vi "work1_GetOrder.vi"() -> ()   [LabVIEW 2026]
panel:
  out "Client order":i32
  out "Order ID":i32
  in  "ID":i32
  in  "stop 2":bool
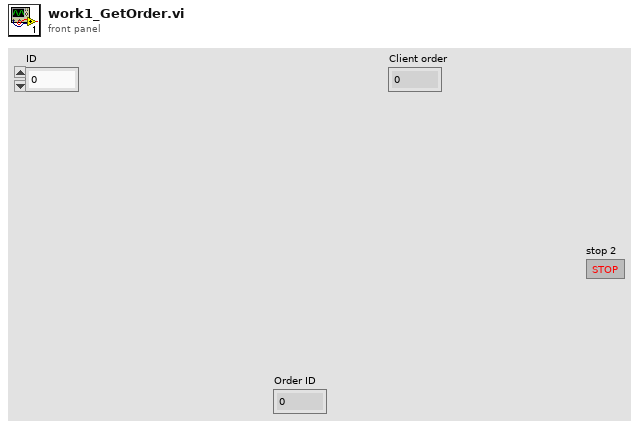
[diagram p1: front panel]
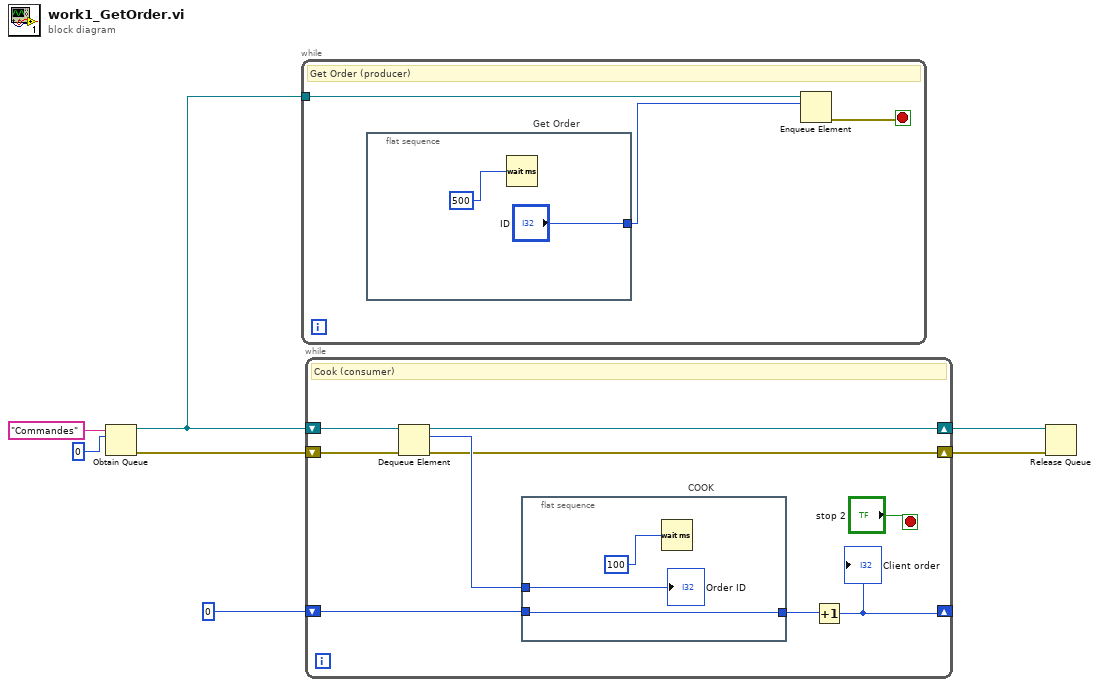
[diagram p0: block diagram]
diagram:
  n1 = Obtain Queue(name (unnamed)="Commandes", element data type=0) -> (queue out=w5:refnum<queue>, error out=w2:errorcluster)  [unwired: 3 in, 1 out]
  n2 = while {
    tunnel: w5 -> [w9]
    stop <- w10 stop-if-true
    # "Get Order (producer)"
    n3 = flat-sequence "Get Order" {
      tunnel: ["ID"] -> w8
      frame #0 {
        n4 = Wait (ms)(milliseconds to wait=500) -> ()  [unwired: 1 out]
      }
    }
    n5 = Enqueue Element(queue=w9, element=w8) -> (error out=w10:errorcluster)  [unwired: 2 in, 2 out]
  }
  n6 = while {
    shift-right: [w19] -> w4
    shift-left: w5 -> [w20]
    shift-right: [w17] -> w3
    shift-left: w2 -> [w16]
    shift-right: [w14] -> _
    shift-left: 0 -> [w15]
    stop <- "stop 2" stop-if-true
    # "Cook (consumer)"
    n7 = Dequeue Element(queue=w20, error in (no error)=w16) -> (queue out=w19:refnum<queue>, element=w18:i32, error out=w17:errorcluster)  [unwired: 1 in, 1 out]
    n8 = flat-sequence "COOK" {
      tunnel: w18 -> [w23]
      tunnel: w15 -> [w22]
      tunnel: [w22] -> w13
      frame #0 {
        n9 = Wait (ms)(milliseconds to wait=100) -> ()  [unwired: 1 out]
        "Order ID" <- w23
      }
    }
    n10 = Increment(x=w13) -> (x+1=w14:i32)
    "Client order" <- w14
  }
  n11 = Release Queue(queue=w4, error in (no error)=w3) -> ()  [unwired: 1 in, 3 out]
